vi "Scripting_ConvertBaseClassToSubClass.vi"(0 "BaseClass":refnum<vi>, 1 "NewBaseClass":path=path "C:/Documents and Settings/Micke/Skrivbord/My Computer/B_class/B.lvclass", 2 "SubClassTemplate":path=path "C:/Program/National Instruments/LabVIEW 8.2/resource/Framework/Providers/Endevo/ClassProviders/Provider_EndevoGOOP300/Templates/SubTemplate/SubTemplate.lvclass", 3 "GOOP4Style":bool, 5 "error in (no error)":errorcluster) -> (19 "error out":errorcluster={"status"=TRUE, "code"=1055, "source"="Property Node in Scripting_ConvertBaseClassToSubClass.vi"})   [LabVIEW 2020]
uses:
  <vilib>/Utility/miscctls.llb/LVPositionTypeDef.ctl
  Provider_EndevoGOOP300/EndevoProviderName.ctl
  Provider_EndevoGOOP300/Templates/EndevoTemplateNames.ctl
  Provider_EndevoGOOP400/EndevoG4ProviderName.ctl
  Provider_EndevoGOOP400/Templates/EndevoG4TemplateNames.ctl
  Provider_LvNativeClass/ClassWriterNative_class/ClassWriterNative.lvclass
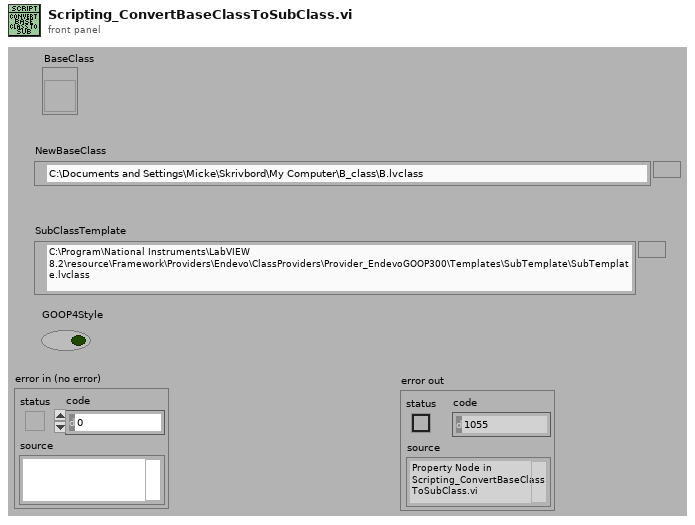
[diagram p1: front panel]
types:
  T1 = cluster{"NewBaseClass":refnum<vi>, "NewBaseCreate ":path, "NewBaseDestroy":path, "NewBaseKernel":path, "NewBaseAttribute":path, "NewBaseClassAttr":path, "NewBaseObjectRef":path, " BaseClass":refnum<vi>, "BaseCreate ":path, "BaseDestroy":path, "BaseKernel":path, "BaseAttribute":path, "BaseClassAttr":path, "BaseClassName":string, "BaseObjectRef":path, "AllBaseClassFiles":path[], "SubNewVi":path, "ObjectRef":refnum<vi>, "BaseNewVi":path, "BaseDeleteVi":path, "SubTemplateKernel":path, "ClassVIs":refnum<vi>[], "SubTemplateClass":refnum<vi>, "BaseTemplateClass":refnum<vi>, "BaseTemplateKernel":path, "BaseAttrRef":refnum<vi>, "BaseClassAttrRef":refnum<vi>, "KernelRef":refnum<vi>, "TemplateVersionUsed":string, "NewBaseNewVI":path, "Singleton":bool, "BaseGetInstance":path, "NewBaseGetInstance":path, "App":refnum<vi>}
  T2 = typedef "LVPositionTypeDef.ctl" = cluster{"Left":i32, "Top":i32}
  T3 = typedef "EndevoTemplateNames.ctl" = enum16{"BaseTemplate", "SubTemplate", "BaseTemplate_4x4x4", "SubTemplate_4x4x4", "SingletonTemplate"}
  T4 = typedef "EndevoProviderName.ctl" = enum16{"EndevoGOOP300"}
  T5 = typedef "EndevoG4TemplateNames.ctl" = enum16{"G4BaseTemplate_Simple_4x4x4", "G4SubTemplate_Simple_4x4x4", "G4BaseTemplate_Simple_6x8x6", "G4SubTemplate_Simple_6x8x6", "G4BaseTemplate_Singleton_4x4x4", "G4SubTemplate_Singleton_4x4x4", "G4BaseTemplate_Singleton_6x8x6", "G4SubTemplate_Singleton_6x8x6", "G4InterfaceTemplate_6x8x6", "G4InterfaceTemplate_4x4x4", "G4BaseTemplate_Simple_5x6x5", "G4BaseTemplate_Singleton_5x6x5", "G4InterfaceTemplate_5x6x5", "G4SubTemplate_Simple_5x6x5", "G4SubTemplate_Singleton_5x6x5"}
  T6 = typedef "EndevoG4ProviderName.ctl" = enum16{"EndevoGOOP400"}
  T7 = cluster{"Major":u16, "Minor":u16, "Fix":u16, "Build":u16}
  T8 = cluster{i32, "WireTermSource":refnum<vi>, "AllWireTerminalDrains":refnum<vi>[]}[]
  T9 = cluster{i32, "AllWireTerminalDrains":refnum<vi>[]}[]
  T10 = typedef "GDSLvCLass_ClassSettingsType.ctl" = cluster{"ClassProviderName":string, "ClassTemplateUsed":string, "ClassTemplateVersion":string, "ClassDescription":string, "PlugIns":T11[], "ConnectorPanePattern":string}
  T11 = typedef "GDSLvClass_PlugIn.ctl" = cluster{"Type":T12, "ID":string, "Version":string, "Path":path, "Name":string, "Data":variant}
  T12 = typedef "GDSLvClass_PlugInTypes.ctl" = enum16{"DesignPattern", "MethodTypes"}
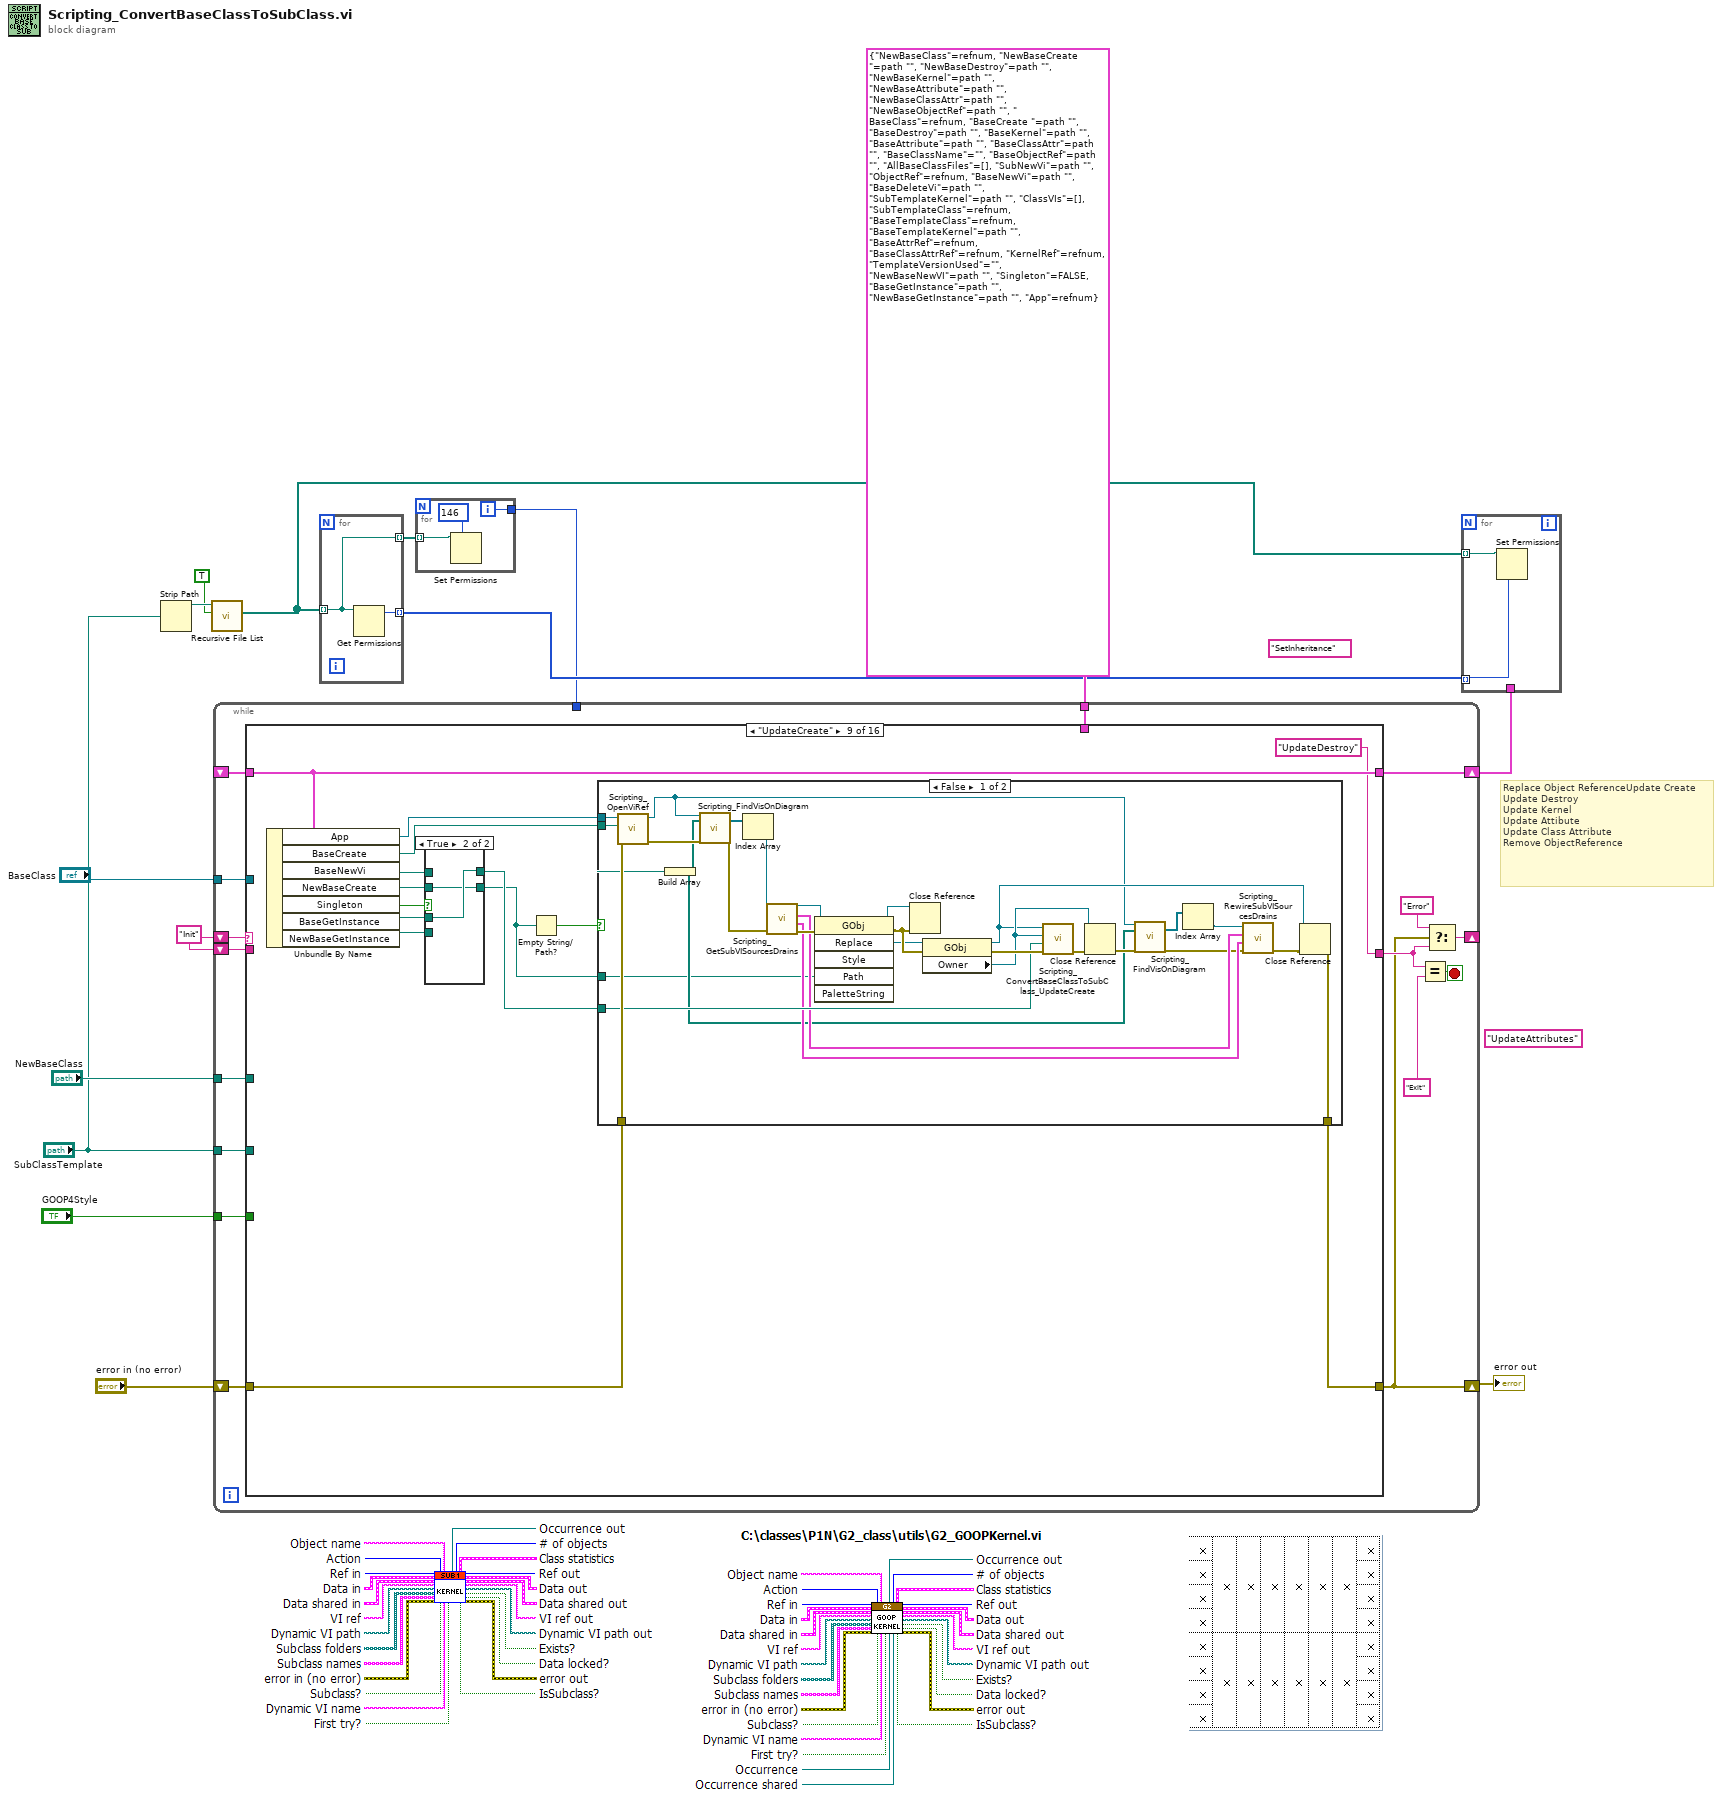
[diagram p0: block diagram]
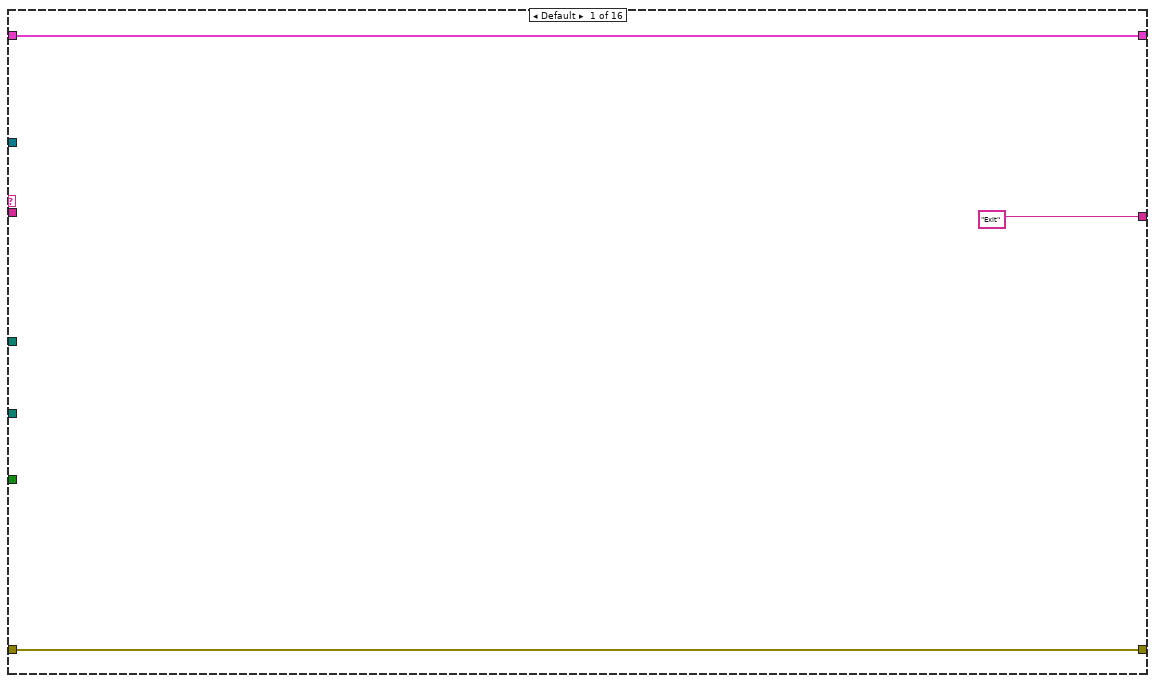
[diagram p2: hidden frame]
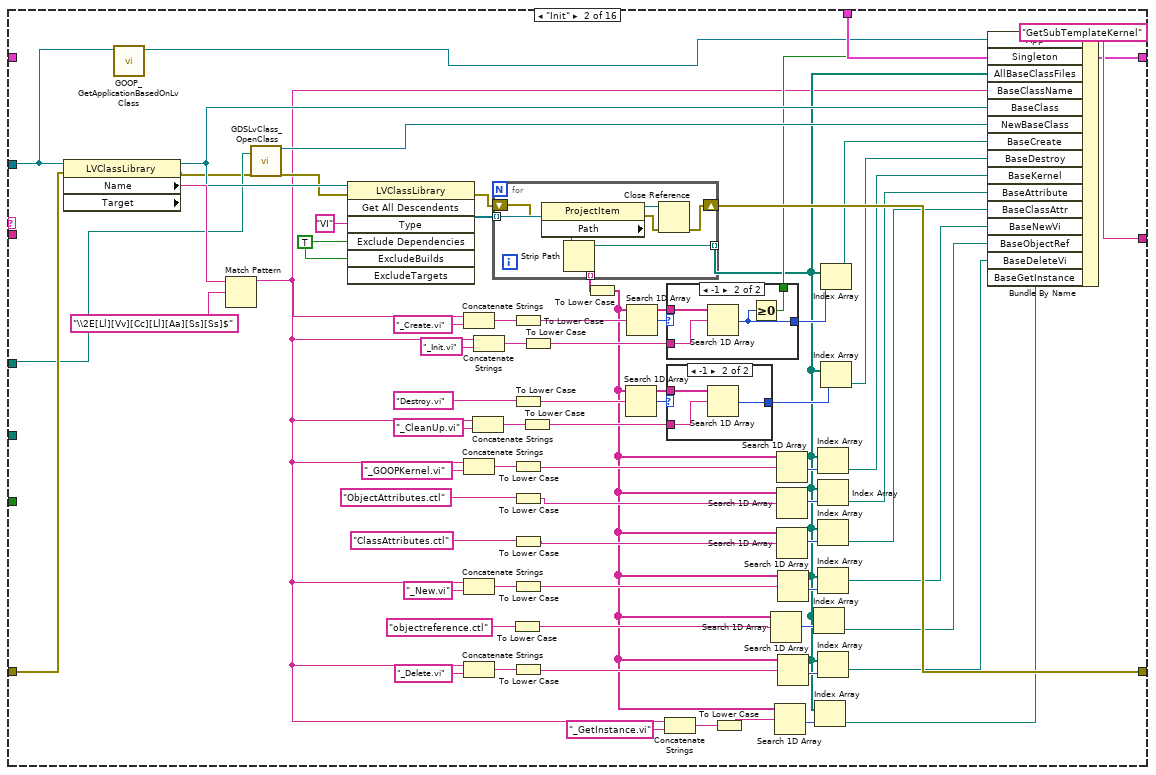
[diagram p3: hidden frame]
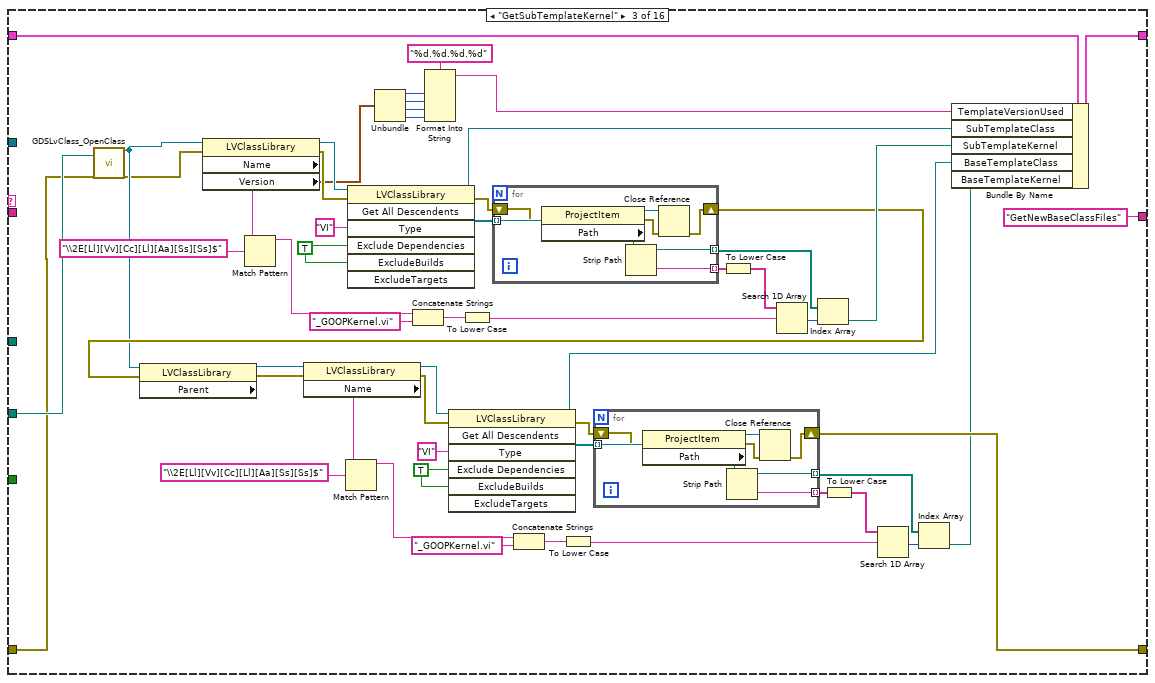
[diagram p6: hidden frame]
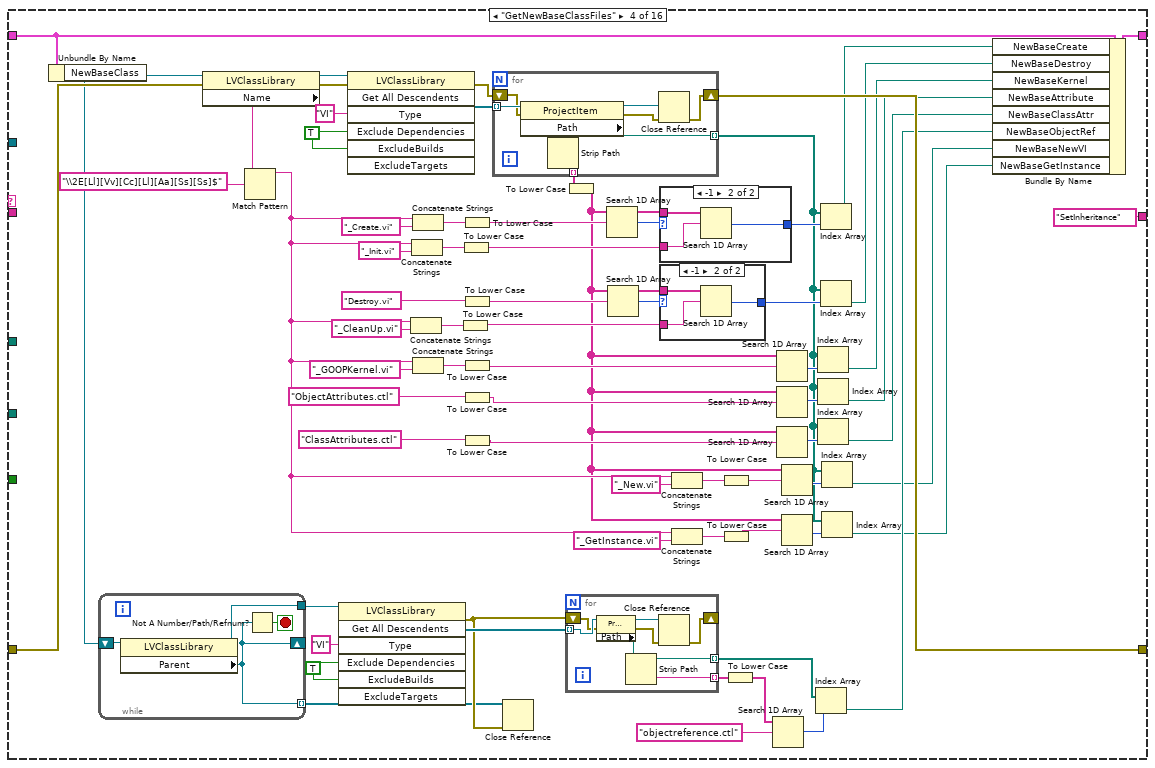
[diagram p7: hidden frame]
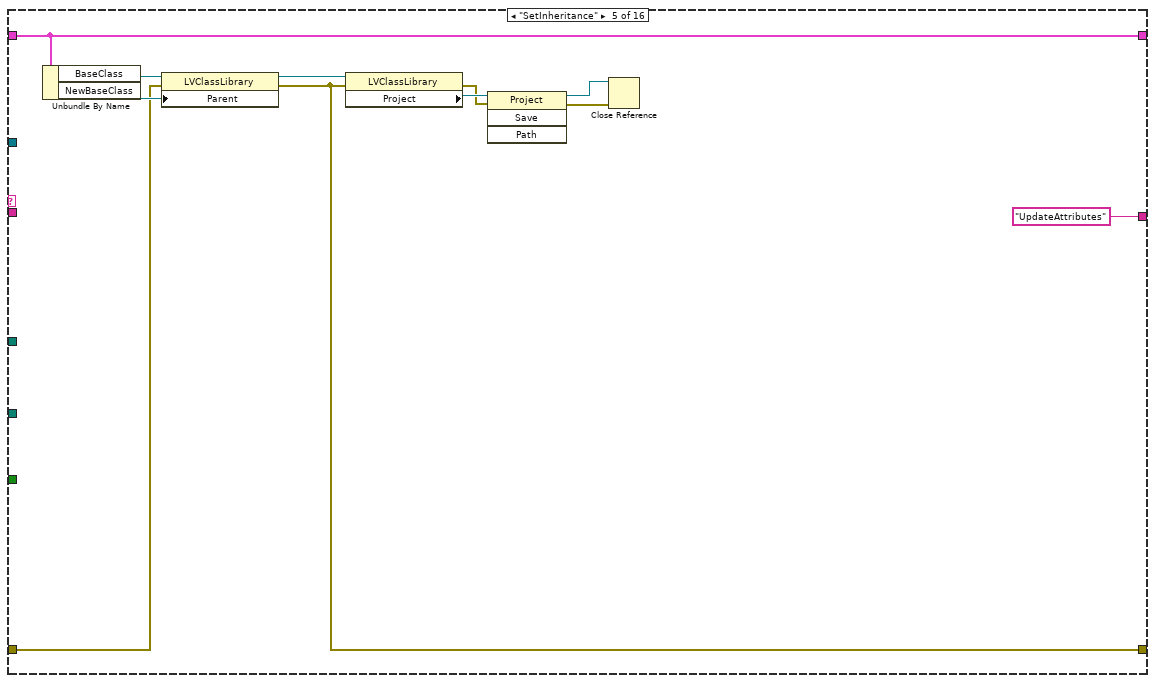
[diagram p10: hidden frame]
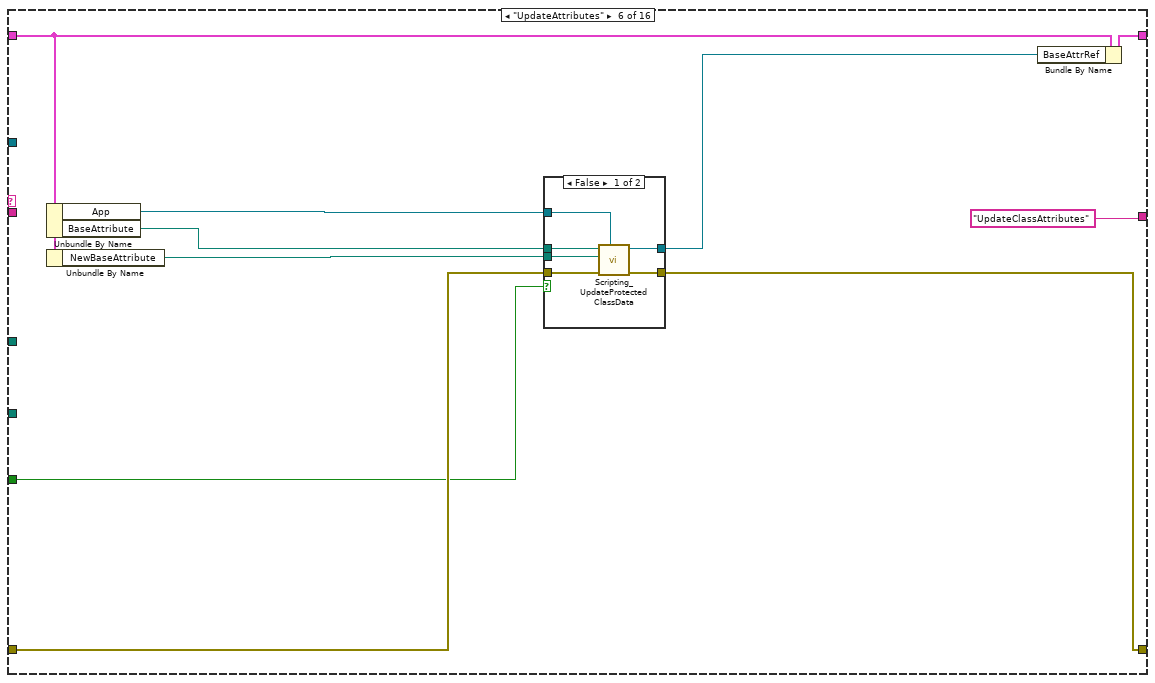
[diagram p11: hidden frame]
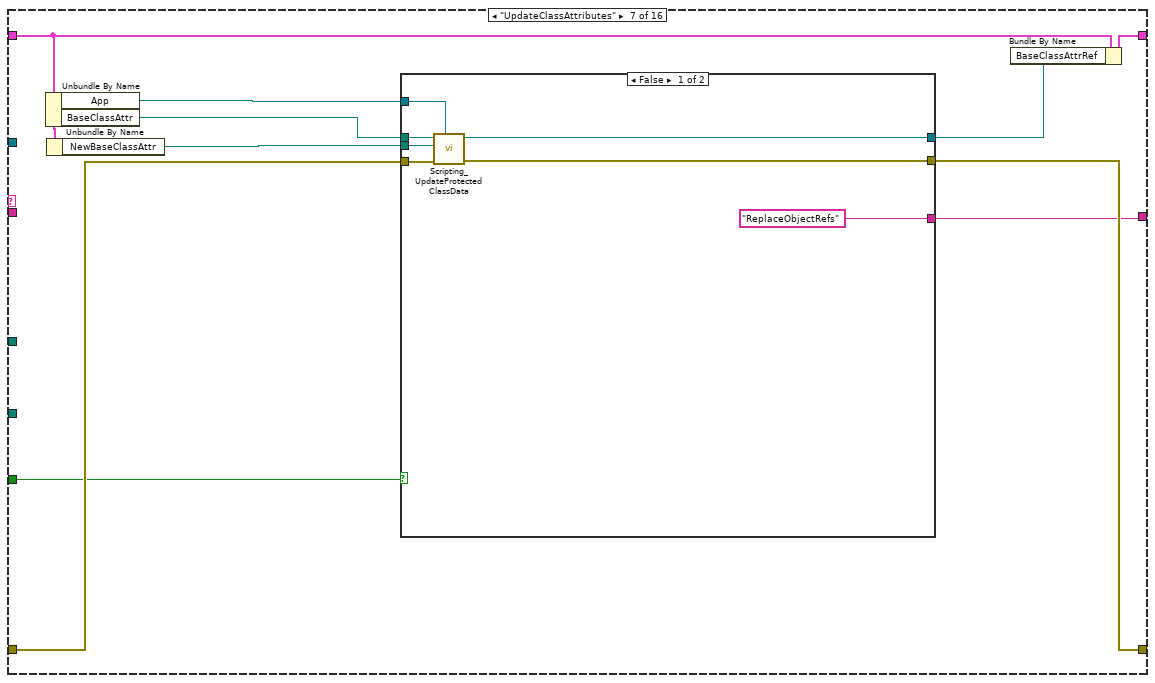
[diagram p13: hidden frame]
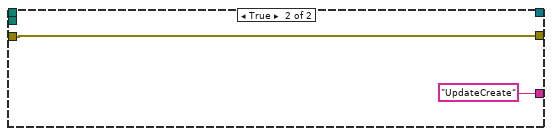
[diagram p14: hidden frame]
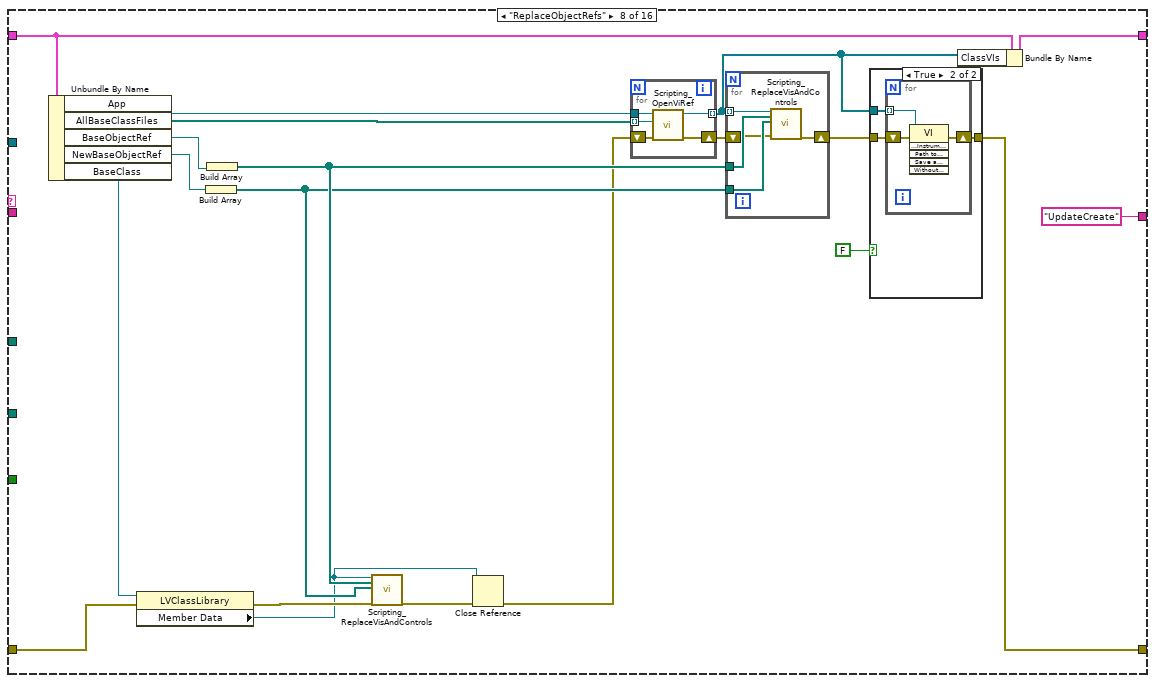
[diagram p15: hidden frame]
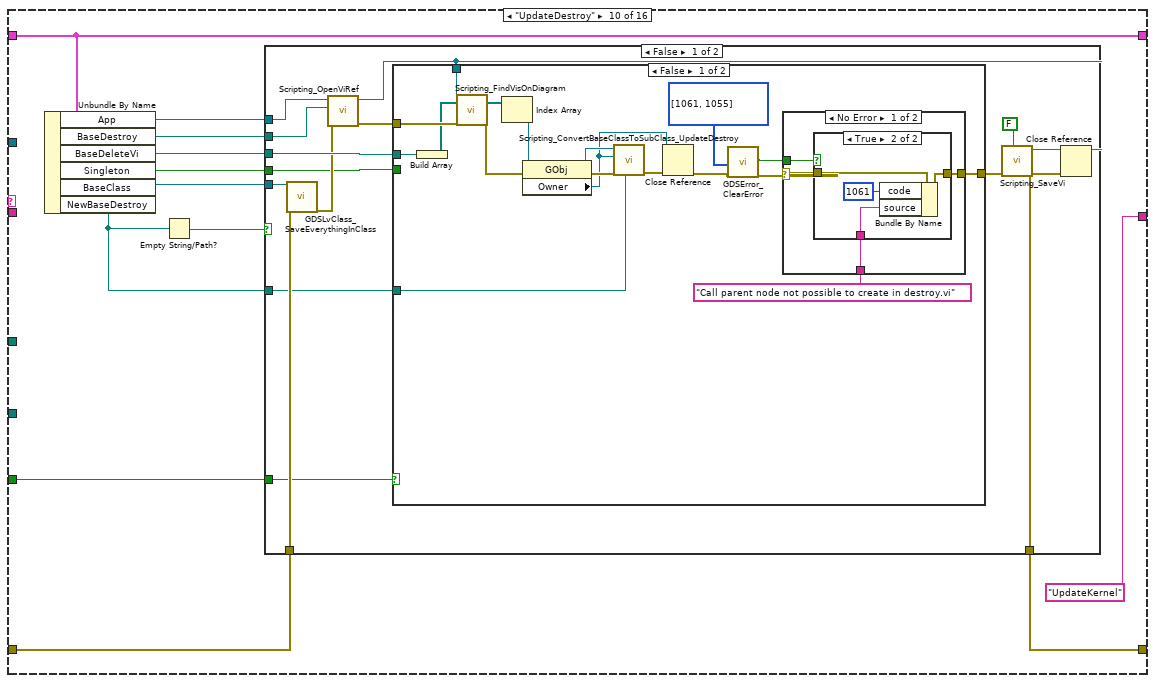
[diagram p19: hidden frame]
diagram:
  (unwired) "SetInheritance"
  (unwired) "UpdateAttributes"
  w10 = "Init"
  # "Replace Object ReferenceUpdate Create\nUpdate Destroy\nUpdate Kernel\nUpdate Attibute\nUpdate Class Attribute\nRemove ObjectReference"
  n1 = Strip Path(path="SubClassTemplate") -> (stripped path=w9:path)  [unwired: 1 out]
  n2 = call <vilib>:"Recursive File List.vi"("Treat LLBs as Folders?"=TRUE, "Folder Path"=w9) -> ("All Files in Dir"=w4:path[])  [unwired: 5 in, 4 out]
  n3 = for {
    tunnel: w4 -> [w16] mode=indexing
    tunnel: [w17] -> w6 mode=indexing
    tunnel: [w16] -> w3 mode=indexing
    n4 = Get Permissions(11:w16) -> (5:w17:i16)  [unwired: 1 in, 4 out]
  }
  n5 = for {
    tunnel: w3 -> [w20] mode=indexing
    tunnel: [w18] -> w5
    i -> [w18]
    n6 = Set Permissions(7:i16 146 ("permissions"), 11:w20) -> ()  [unwired: 3 in, 2 out]
  }
  n7 = while {
    shift-right: [w29] -> w14
    shift-left: "error in (no error)" -> [w36]
    shift-right: [w34] -> _
    shift-left: w10 -> [w35]
    shift-right: [w28] -> w7
    shift-left: _ -> [w27]
    tunnel: "BaseClass" -> [w26]
    tunnel: T1 {"NewBaseClass"=refnum, "NewBaseCreate "=path "", "NewBaseDestroy"=path "", "NewBaseKernel"=path "", "NewBaseAttribute"=path "", "NewBaseClassAttr"=path "", "NewBaseObjectRef"=path "", " BaseClass"=refnum, "BaseCreate "=path "", "BaseDestroy"=path "", "BaseKernel"=path "", "BaseAttribute"=path "", "BaseClassAttr"=path "", "BaseClassName"="", "BaseObjectRef"=path "", "AllBaseClassFiles"=[], "SubNewVi"=path "", "ObjectRef"=refnum, "BaseNewVi"=path "", "BaseDeleteVi"=path "", "SubTemplateKernel"=path "", "ClassVIs"=[], "SubTemplateClass"=refnum, "BaseTemplateClass"=refnum, "BaseTemplateKernel"=path "", "BaseAttrRef"=refnum, "BaseClassAttrRef"=refnum, "KernelRef"=refnum, "TemplateVersionUsed"="", "NewBaseNewVI"=path "", "Singleton"=FALSE, "BaseGetInstance"=path "", "NewBaseGetInstance"=path "", "App"=refnum} -> [w25]
    tunnel: "NewBaseClass" -> [w24]
    tunnel: "SubClassTemplate" -> [w23]
    shift-left: w10 -> [w22]
    tunnel: w5 -> [_]
    tunnel: "GOOP4Style" -> [w21]
    stop <- w33 stop-if-true
    n8 = case shown="\"UpdateCreate\"" w35 {
      tunnel: w36 -> [w39 w77 w137 w236 w299 w310 w325 w347 w387 w429 w503 w643 w673 w715 w760 w770]
      tunnel: [w39 w102 w141 w255 w292 w306 w324 w344 w386 w427 w502 w642 w672 w699 w759 w770] -> w29
      tunnel: ["Exit" "GetSubTemplateKernel" "GetNewBaseClassFiles" "SetInheritance" "UpdateAttributes" "UpdateClassAttributes" w321 "UpdateCreate" "UpdateDestroy" "UpdateKernel" w504 "UpdateClassInfo" "RemoveObjectRef_And_SaveFiles" "UpdateAllDerivedClasses" "CloseReferences" "Exit"] -> w30
      tunnel: [w37 w110 w181 w265 w301 w307 w328 w352 w389 w434 w500 w640 w670 w714 w762 w768] -> w28
      tunnel: w27 -> [w37 _ w169 w237 w301 w308 w329 w353 w389 w434 w501 w640 w670 w714 w762 w768]
      tunnel: w26 -> [_ w41 _ _ _ _ _ _ _ _ _ _ _ _ w758 _]
      tunnel: w25 -> [_ w84 _ _ _ _ _ _ _ _ _ _ _ _ _ _]
      tunnel: w24 -> [_ w65 _ _ _ _ _ _ _ _ _ _ _ _ _ _]
      tunnel: w23 -> [_ _ w166 _ _ _ _ _ _ _ _ _ _ _ _ _]
      tunnel: w22 -> [_ _ _ _ _ _ _ _ _ _ _ _ _ _ _ w769]
      tunnel: w21 -> [_ _ _ _ _ w304 w322 _ _ w428 w499 w644 w663 w697 w757 _]
      frame Default {
      }
      frame "Init" {
        w61 = TRUE ("ExcludeDependencies")
        n9 = property class="LVClassLibrary" props=["Name", "Target"](reference=w41, error in=w77) -> (reference out=w75:refnum<vi>, error out=w64:errorcluster, "Name"=w76:string)  [unwired: 1 out]
        n10 = call "GOOP_GetApplicationBasedOnLvClass.vi"("LVClassLibrary in"=w41) -> ("Application out"=w40:refnum<vi>)  [unwired: 9 in, 1 out]
        n11 = Match Pattern(string=w76, regular expression="\\2E[Ll][Vv][Cc][Ll][Aa][Ss][Ss]$") -> (before substring=w43:string)  [unwired: 1 in, 3 out]
        n12 = call "GDSLvClass_OpenClass.vi"("ClassToOpen"=w65, "error in (no error)"=w64) -> ("LVClass.Open"=w62:refnum<vi>, "error out"=w63:errorcluster)  [unwired: 16 in]
        n13 = invoke class="LVClassLibrary" method="Get All Descendents"(reference=w75, error in=w63, "Type"="VI", "Exclude Dependencies"=w61, "ExcludeBuilds"=w61) -> (error out=w107:errorcluster, "All Descendents"=w108:refnum<vi>[])  [unwired: 2 in, 5 out]
        n14 = Concatenate Strings(w43, "_Create.vi" ("string")) -> (w104:string)
        n15 = Concatenate Strings(w43, "_GOOPKernel.vi" ("string")) -> (w98:string)
        n16 = Concatenate Strings(w43, "_New.vi" ("string")) -> (w81:string)
        n17 = Concatenate Strings(w43, "_Delete.vi" ("string")) -> (w69:string)
        n18 = Concatenate Strings(w43, "_CleanUp.vi" ("string")) -> (w59:string)
        n19 = Concatenate Strings(w43, "_Init.vi" ("string")) -> (w60:string)
        n20 = for {
          tunnel: w108 -> [w127] mode=indexing
          shift-right: [w123] -> w102
          shift-left: w107 -> [w124]
          tunnel: [w122] -> w45 mode=indexing
          tunnel: [w121] -> w105 mode=indexing
          n21 = property class="ProjectItem"(reference=w127, error in=w124) -> (reference out=w126:refnum<vi>, error out=w125:errorcluster, "Path"=w122:path)
          n22 = Strip Path(path=w122) -> (name=w121:string)  [unwired: 1 out]
          n23 = Close Reference(reference=w126, error in (no error)=w125) -> (error out=w123:errorcluster)
        }
        n24 = To Lower Case(string="objectreference.ctl" ("element")) -> (all lower case string=w73:string)
        n25 = To Lower Case(string=w104) -> (all lower case string=w103:string)
        n26 = To Lower Case(string="Destroy.vi") -> (all lower case string=w100:string)
        n27 = To Lower Case(string=w98) -> (all lower case string=w96:string)
        n28 = To Lower Case(string="ObjectAttributes.ctl") -> (all lower case string=w91:string)
        n29 = To Lower Case(string="ClassAttributes.ctl") -> (all lower case string=w88:string)
        n30 = To Lower Case(string=w81) -> (all lower case string=w82:string)
        n31 = To Lower Case(string=w69) -> (all lower case string=w67:string)
        n32 = To Lower Case(string=w59) -> (all lower case string=w57:string)
        n33 = To Lower Case(string=w60) -> (all lower case string=w58:string)
        n34 = To Lower Case(string=w105) -> (all lower case string=w44:string[])
        n35 = Search 1D Array(1D array=w44, element=w100) -> (index of element=w54:i32)  [unwired: 1 in]
        n36 = Search 1D Array(1D array=w44, element=w103) -> (index of element=w56:i32)  [unwired: 1 in]
        n37 = Concatenate Strings(w43, "_GetInstance.vi" ("string")) -> (w48:string)
        n38 = case shown="-1" w56 {
          selector: w56 -> [w116 _]
          tunnel: w44 -> [_ w120]
          tunnel: w58 -> [_ w119]
          tunnel: [w116 w118] -> w55
          tunnel: [_ w117] -> w50
          frame 0, Default {
          }
          frame -1 {
            n39 = Search 1D Array(1D array=w120, element=w119) -> (index of element=w118:i32)  [unwired: 1 in]
            n40 = Greater Or Equal To 0?(x=w118) -> (x >= 0?=w117:bool)
          }
        }
        n41 = case shown="-1" w54 {
          selector: w54 -> [w112 _]
          tunnel: w44 -> [_ w115]
          tunnel: w57 -> [_ w114]
          tunnel: [w112 w113] -> w53
          frame 0, Default {
          }
          frame -1 {
            n42 = Search 1D Array(1D array=w115, element=w114) -> (index of element=w113:i32)  [unwired: 1 in]
          }
        }
        n43 = To Lower Case(string=w48) -> (all lower case string=w46:string)
        n44 = Search 1D Array(1D array=w44, element=w73) -> (index of element=w74:i32)  [unwired: 1 in]
        n45 = Search 1D Array(1D array=w44, element=w46) -> (index of element=w47:i32)  [unwired: 1 in]
        n46 = Search 1D Array(1D array=w44, element=w96) -> (index of element=w95:i32)  [unwired: 1 in]
        n47 = Search 1D Array(1D array=w44, element=w91) -> (index of element=w90:i32)  [unwired: 1 in]
        n48 = Search 1D Array(1D array=w44, element=w88) -> (index of element=w89:i32)  [unwired: 1 in]
        n49 = Search 1D Array(1D array=w44, element=w82) -> (index of element=w79:i32)  [unwired: 1 in]
        n50 = Search 1D Array(1D array=w44, element=w67) -> (index of element=w68:i32)  [unwired: 1 in]
        n51 = Index Array(array=w45, index=w74) -> (element=w71:path)
        n52 = Index Array(array=w45, index=w47) -> (element=w42:path)
        n53 = Index Array(array=w45, index=w95) -> (element=w87:path)
        n54 = Index Array(array=w45, index=w90) -> (element=w86:path)
        n55 = Index Array(array=w45, index=w89) -> (element=w85:path)
        n56 = Index Array(array=w45, index=w79) -> (element=w78:path)
        n57 = Index Array(array=w45, index=w68) -> (element=w66:path)
        n58 = Index Array(array=w45, index=w55) -> (element=w99:path)
        n59 = Index Array(array=w45, index=w53) -> (element=w94:path)
        n60 = Bundle By Name(cluster=w84, "App"=w40, "Singleton"=w50, "AllBaseClassFiles"=w45, "BaseClassName"=w43, "BaseClass"=w75, "NewBaseClass"=w62, "BaseCreate"=w99, "BaseDestroy"=w94, "BaseKernel"=w87, "BaseAttribute"=w86, "BaseClassAttr"=w85, "BaseNewVi"=w78, "BaseObjectRef"=w71, "BaseDeleteVi"=w66, "BaseGetInstance"=w42) -> (w110:T1)
      }
      frame "GetSubTemplateKernel" {
        w135 = TRUE ("ExcludeDependencies")
        w136 = TRUE ("ExcludeDependencies")
        n61 = call "GDSLvClass_OpenClass.vi"("ClassToOpen"=w166, "error in (no error)"=w137) -> ("LVClass.Open"=w159:refnum<vi>, "error out"=w138:errorcluster)  [unwired: 16 in]
        n62 = property class="LVClassLibrary"(reference=w159, error in=w138) -> (reference out=w176:refnum<vi>, error out=w177:errorcluster, "Name"=w168:string, "Version"=w129:T7)
        n63 = Match Pattern(string=w168, regular expression="\\2E[Ll][Vv][Cc][Ll][Aa][Ss][Ss]$") -> (before substring=w165:string)  [unwired: 1 in, 3 out]
        n64 = invoke class="LVClassLibrary" method="Get All Descendents"(reference=w176, error in=w177, "Type"="VI", "Exclude Dependencies"=w135, "ExcludeBuilds"=w135) -> (reference out=w161:refnum<vi>, error out=w178:errorcluster, "All Descendents"=w179:refnum<vi>[])  [unwired: 2 in, 4 out]
        n65 = Unbundle(w129) -> ("Major"=w134:u16, "Minor"=w133:u16, "Fix"=w132:u16, "Build"=w131:u16)
        n66 = Concatenate Strings(w165, "_GOOPKernel.vi" ("string")) -> (w174:string)
        n67 = Format Into String(format string="%d.%d.%d.%d", w134, w133, w132, w131) -> (resulting string=w128:string)  [unwired: 2 in, 1 out]
        n68 = To Lower Case(string=w174) -> (all lower case string=w172:string)
        n69 = for {
          tunnel: w179 -> [w195] mode=indexing
          shift-right: [w191] -> w160
          shift-left: w178 -> [w192]
          tunnel: [w190] -> w164 mode=indexing
          tunnel: [w189] -> w175 mode=indexing
          n70 = property class="ProjectItem"(reference=w195, error in=w192) -> (reference out=w194:refnum<vi>, error out=w193:errorcluster, "Path"=w190:path)
          n71 = Strip Path(path=w190) -> (name=w189:string)  [unwired: 1 out]
          n72 = Close Reference(reference=w194, error in (no error)=w193) -> (error out=w191:errorcluster)
        }
        n73 = property class="LVClassLibrary"(reference=w159, error in=w160) -> (error out=w143:errorcluster, "Parent"=w144:refnum<vi>)  [unwired: 1 out]
        n74 = property class="LVClassLibrary"(reference=w144, error in=w143) -> (reference out=w149:refnum<vi>, error out=w148:errorcluster, "Name"=w155:string)
        n75 = Match Pattern(string=w155, regular expression="\\2E[Ll][Vv][Cc][Ll][Aa][Ss][Ss]$") -> (before substring=w156:string)  [unwired: 1 in, 3 out]
        n76 = invoke class="LVClassLibrary" method="Get All Descendents"(reference=w149, error in=w148, "Type"="VI", "Exclude Dependencies"=w136, "ExcludeBuilds"=w136) -> (reference out=w142:refnum<vi>, error out=w147:errorcluster, "All Descendents"=w146:refnum<vi>[])  [unwired: 2 in, 4 out]
        n77 = Concatenate Strings(w156, "_GOOPKernel.vi" ("string")) -> (w151:string)
        n78 = To Lower Case(string=w151) -> (all lower case string=w153:string)
        n79 = for {
          tunnel: w146 -> [w188] mode=indexing
          shift-right: [w184] -> w141
          shift-left: w147 -> [w185]
          tunnel: [w183] -> w157 mode=indexing
          tunnel: [w182] -> w150 mode=indexing
          n80 = property class="ProjectItem"(reference=w188, error in=w185) -> (reference out=w187:refnum<vi>, error out=w186:errorcluster, "Path"=w183:path)
          n81 = Strip Path(path=w183) -> (name=w182:string)  [unwired: 1 out]
          n82 = Close Reference(reference=w187, error in (no error)=w186) -> (error out=w184:errorcluster)
        }
        n83 = To Lower Case(string=w175) -> (all lower case string=w163:string[])
        n84 = Search 1D Array(1D array=w163, element=w172) -> (index of element=w171:i32)  [unwired: 1 in]
        n85 = Index Array(array=w164, index=w171) -> (element=w170:path)
        n86 = To Lower Case(string=w150) -> (all lower case string=w158:string[])
        n87 = Search 1D Array(1D array=w158, element=w153) -> (index of element=w154:i32)  [unwired: 1 in]
        n88 = Index Array(array=w157, index=w154) -> (element=w140:path)
        n89 = Bundle By Name(cluster=w169, "TemplateVersionUsed"=w128, "SubTemplateClass"=w161, "SubTemplateKernel"=w170, "BaseTemplateClass"=w142, "BaseTemplateKernel"=w140) -> (w181:T1)
      }
      frame "GetNewBaseClassFiles" {
        w221 = TRUE ("ExcludeDependencies")
        w222 = TRUE ("ExcludeDependencies")
        n90 = Unbundle By Name(w237) -> ("NewBaseClass"=w234:refnum<vi>)
        n91 = while {
          shift-right: [w282] -> _
          shift-left: w234 -> [w283]
          tunnel: [w282] -> w204 mode=indexing
          tunnel: [w281] -> w232
          stop <- w284 stop-if-true
          n92 = property class="LVClassLibrary"(reference=w283) -> (reference out=w281:refnum<vi>, "Parent"=w282:refnum<vi>)  [unwired: 1 in, 1 out]
          n93 = Not A Number/Path/Refnum?(number/path/refnum=w282) -> (NaN/Path/Refnum?=w284:bool)
        }
        n94 = property class="LVClassLibrary"(reference=w234, error in=w236) -> (reference out=w260:refnum<vi>, error out=w261:errorcluster, "Name"=w235:string)
        n95 = Match Pattern(string=w235, regular expression="\\2E[Ll][Vv][Cc][Ll][Aa][Ss][Ss]$") -> (before substring=w201:string)  [unwired: 1 in, 3 out]
        n96 = invoke class="LVClassLibrary" method="Get All Descendents"(reference=w232, "Type"="VI", "Exclude Dependencies"=w222, "ExcludeBuilds"=w222) -> (error out=w205:errorcluster, "All Descendents"=w231:refnum<vi>[])  [unwired: 3 in, 5 out]
        n97 = invoke class="LVClassLibrary" method="Get All Descendents"(reference=w260, error in=w261, "Type"="VI", "Exclude Dependencies"=w221, "ExcludeBuilds"=w221) -> (error out=w262:errorcluster, "All Descendents"=w263:refnum<vi>[])  [unwired: 2 in, 5 out]
        n98 = Concatenate Strings(w201, "_CleanUp.vi" ("string")) -> (w210:string)
        n99 = Concatenate Strings(w201, "_Init.vi" ("string")) -> (w211:string)
        n100 = Concatenate Strings(w201, "_Create.vi" ("string")) -> (w257:string)
        n101 = Concatenate Strings(w201, "_GOOPKernel.vi" ("string")) -> (w251:string)
        n102 = To Lower Case(string=w210) -> (all lower case string=w206:string)
        n103 = To Lower Case(string=w211) -> (all lower case string=w207:string)
        n104 = To Lower Case(string=w257) -> (all lower case string=w256:string)
        n105 = To Lower Case(string="Destroy.vi") -> (all lower case string=w253:string)
        n106 = To Lower Case(string=w251) -> (all lower case string=w249:string)
        n107 = To Lower Case(string="ObjectAttributes.ctl") -> (all lower case string=w244:string)
        n108 = To Lower Case(string="ClassAttributes.ctl") -> (all lower case string=w241:string)
        n109 = for {
          tunnel: w263 -> [w291] mode=indexing
          shift-right: [w287] -> w255
          shift-left: w262 -> [w288]
          tunnel: [w286] -> w199 mode=indexing
          tunnel: [w285] -> w258 mode=indexing
          n110 = property class="ProjectItem"(reference=w291, error in=w288) -> (reference out=w290:refnum<vi>, error out=w289:errorcluster, "Path"=w286:path)
          n111 = Strip Path(path=w286) -> (name=w285:string)  [unwired: 1 out]
          n112 = Close Reference(reference=w290, error in (no error)=w289) -> (error out=w287:errorcluster)
        }
        n113 = Close Reference(reference=w204, error in (no error)=w205) -> ()  [unwired: 1 out]
        n114 = To Lower Case(string=w258) -> (all lower case string=w198:string[])
        n115 = for {
          tunnel: w231 -> [w280] mode=indexing
          shift-right: [w276] -> _
          shift-left: w205 -> [w277]
          tunnel: [w275] -> w226 mode=indexing
          tunnel: [w274] -> w230 mode=indexing
          n116 = property class="ProjectItem"(reference=w280, error in=w277) -> (reference out=w279:refnum<vi>, error out=w278:errorcluster, "Path"=w275:path)
          n117 = Strip Path(path=w275) -> (name=w274:string)  [unwired: 1 out]
          n118 = Close Reference(reference=w279, error in (no error)=w278) -> (error out=w276:errorcluster)
        }
        n119 = Search 1D Array(1D array=w198, element=w256) -> (index of element=w215:i32)  [unwired: 1 in]
        n120 = Search 1D Array(1D array=w198, element=w253) -> (index of element=w213:i32)  [unwired: 1 in]
        n121 = case shown="-1" w215 {
          selector: w215 -> [w270 _]
          tunnel: w198 -> [_ w273]
          tunnel: w207 -> [_ w272]
          tunnel: [w270 w271] -> w214
          frame 0, Default {
          }
          frame -1 {
            n122 = Search 1D Array(1D array=w273, element=w272) -> (index of element=w271:i32)  [unwired: 1 in]
          }
        }
        n123 = case shown="-1" w213 {
          selector: w213 -> [w266 _]
          tunnel: w198 -> [_ w269]
          tunnel: w206 -> [_ w268]
          tunnel: [w266 w267] -> w212
          frame 0, Default {
          }
          frame -1 {
            n124 = Search 1D Array(1D array=w269, element=w268) -> (index of element=w267:i32)  [unwired: 1 in]
          }
        }
        n125 = Concatenate Strings(w201, "_New.vi" ("string")) -> (w219:string)
        n126 = Concatenate Strings(w201, "_GetInstance.vi" ("string")) -> (w202:string)
        n127 = To Lower Case(string=w219) -> (all lower case string=w220:string)
        n128 = To Lower Case(string=w202) -> (all lower case string=w197:string)
        n129 = To Lower Case(string=w230) -> (all lower case string=w224:string[])
        n130 = Search 1D Array(1D array=w224, element="objectreference.ctl") -> (index of element=w227:i32)  [unwired: 1 in]
        n131 = Search 1D Array(1D array=w198, element=w249) -> (index of element=w248:i32)  [unwired: 1 in]
        n132 = Search 1D Array(1D array=w198, element=w244) -> (index of element=w243:i32)  [unwired: 1 in]
        n133 = Search 1D Array(1D array=w198, element=w241) -> (index of element=w242:i32)  [unwired: 1 in]
        n134 = Search 1D Array(1D array=w198, element=w220) -> (index of element=w217:i32)  [unwired: 1 in]
        n135 = Search 1D Array(1D array=w198, element=w197) -> (index of element=w200:i32)  [unwired: 1 in]
        n136 = Index Array(array=w226, index=w227) -> (element=w225:path)
        n137 = Index Array(array=w199, index=w248) -> (element=w240:path)
        n138 = Index Array(array=w199, index=w243) -> (element=w239:path)
        n139 = Index Array(array=w199, index=w242) -> (element=w238:path)
        n140 = Index Array(array=w199, index=w214) -> (element=w252:path)
        n141 = Index Array(array=w199, index=w212) -> (element=w247:path)
        n142 = Index Array(array=w199, index=w217) -> (element=w216:path)
        n143 = Index Array(array=w199, index=w200) -> (element=w196:path)
        n144 = Bundle By Name(cluster=w237, "NewBaseCreate"=w252, "NewBaseDestroy"=w247, "NewBaseKernel"=w240, "NewBaseAttribute"=w239, "NewBaseClassAttr"=w238, "NewBaseObjectRef"=w225, "NewBaseNewVI"=w216, "NewBaseGetInstance"=w196) -> (w265:T1)
      }
      frame "SetInheritance" {
        n145 = Unbundle By Name(w301) -> ("BaseClass"=w302:refnum<vi>, "NewBaseClass"=w300:refnum<vi>)
        n146 = property class="LVClassLibrary"(reference=w302, error in=w299, "Parent"=w300) -> (reference out=w297:refnum<vi>, error out=w292:errorcluster)
        n147 = property class="LVClassLibrary"(reference=w297, error in=w292) -> (error out=w293:errorcluster, "Project"=w296:refnum<vi>)  [unwired: 1 out]
        n148 = invoke class="Project" method="Save"(reference=w296, error in=w293) -> (reference out=w294:refnum<vi>, error out=w295:errorcluster)  [unwired: 2 in, 2 out]
        n149 = Close Reference(reference=w294, error in (no error)=w295) -> ()  [unwired: 1 out]
      }
      frame "UpdateAttributes" {
        n150 = Unbundle By Name(w308) -> ("App"=w303:refnum<vi>, "BaseAttribute"=w311:path)
        n151 = Unbundle By Name(w308) -> ("NewBaseAttribute"=w309:path)
        n152 = case shown="False" w304 {
          tunnel: w311 -> [w318 _]
          tunnel: w310 -> [w317 w319]
          tunnel: w309 -> [w316 _]
          tunnel: [w315 w319] -> w306
          tunnel: [w314 _] -> w305
          tunnel: w303 -> [w313 _]
          frame False {
            n153 = call "Scripting_UpdateProtectedClassData.vi"("AppRef"=w313, "error in (no error)"=w317, "NewBaseAttribute"=w316, "BaseAttribute"=w318) -> ("error out"=w315:errorcluster, "BaseAttributeReference"=w314:refnum<vi>)  [unwired: 6 in]
          }
          frame True {
          }
        }
        n154 = Bundle By Name(cluster=w308, "BaseAttrRef"=w305) -> (w307:T1)
      }
      frame "UpdateClassAttributes" {
        n155 = Unbundle By Name(w329) -> ("App"=w320:refnum<vi>, "BaseClassAttr"=w327:path)
        n156 = Unbundle By Name(w329) -> ("NewBaseClassAttr"=w326:path)
        n157 = case shown="False" w322 {
          tunnel: w327 -> [w336 _]
          tunnel: w326 -> [w335 _]
          tunnel: w325 -> [w334 w338]
          tunnel: [w333 w338] -> w324
          tunnel: [w332 _] -> w323
          tunnel: ["ReplaceObjectRefs" "UpdateCreate"] -> w321
          tunnel: w320 -> [w330 _]
          frame False {
            n158 = call "Scripting_UpdateProtectedClassData.vi"("AppRef"=w330, "error in (no error)"=w334, "NewBaseAttribute"=w335, "BaseAttribute"=w336) -> ("error out"=w333:errorcluster, "BaseAttributeReference"=w332:refnum<vi>)  [unwired: 6 in]
          }
          frame True {
          }
        }
        n159 = Bundle By Name(cluster=w329, "BaseClassAttrRef"=w323) -> (w328:T1)
      }
      frame "ReplaceObjectRefs" {
        n160 = Unbundle By Name(w353) -> ("App"=w339:refnum<vi>, "AllBaseClassFiles"=w350:path[], "BaseObjectRef"=w357:path, "NewBaseObjectRef"=w356:path, "BaseClass"=w348:refnum<vi>)
        n161 = property class="LVClassLibrary"(reference=w348, error in=w347) -> (error out=w346:errorcluster, "Member Data"=w343:refnum<vi>)  [unwired: 1 out]
        n162 = Build Array(w356) -> (w354:path[])
        n163 = Build Array(w357) -> (w355:path[])
        n164 = call "Scripting_ReplaceVisAndControls.vi"("ViRef"=w343, "OldVIsAndControls"=w355, "NewVIsAndControls"=w354, "error in (no error)"=w346) -> ("error out"=w340:errorcluster)  [unwired: 14 in, 1 out]
        n165 = Close Reference(reference=w343, error in (no error)=w340) -> (error out=w345:errorcluster)
        n166 = for {
          shift-right: [w370] -> w342
          shift-left: w345 -> [w369]
          tunnel: w350 -> [w368] mode=indexing
          tunnel: [w367] -> w349 mode=indexing
          tunnel: w339 -> [w366]
          n167 = call "Scripting_OpenViRef.vi"("error in"=w369, "ViPath/ViName/Viref"=w368, "AppRef"=w366) -> ("error out"=w370:errorcluster, "vi reference"=w367:refnum<vi>)  [unwired: 6 in, 1 out]
        }
        n168 = for {
          shift-right: [w375] -> w351
          shift-left: w342 -> [w372]
          tunnel: w355 -> [w374]
          tunnel: w354 -> [w373]
          tunnel: w349 -> [w371] mode=indexing
          n169 = call "Scripting_ReplaceVisAndControls.vi"("ViRef"=w371, "OldVIsAndControls"=w374, "NewVIsAndControls"=w373, "error in (no error)"=w372) -> ("error out"=w375:errorcluster)  [unwired: 14 in, 1 out]
        }
        n170 = case shown="True" FALSE {
          tunnel: w351 -> [w359 w362]
          tunnel: w349 -> [_ w361]
          tunnel: [w359 w360] -> w344
          frame False {
          }
          frame True {
            n171 = for {
              shift-right: [w364] -> w360
              shift-left: w362 -> [w365]
              tunnel: w361 -> [w363] mode=indexing
              n172 = invoke class="VI" method="Save.Instrument"(reference=w363, error in=w365) -> (error out=w364:errorcluster)  [unwired: 4 in, 5 out]
            }
          }
        }
        n173 = Bundle By Name(cluster=w353, "ClassVIs"=w349) -> (w352:T1)
      }
      frame "UpdateCreate" {
        n174 = Unbundle By Name(w389) -> ("App"=w379:refnum<vi>, "BaseCreate"=w388:path, "BaseNewVi"=w384:path, "NewBaseCreate"=w383:path, "Singleton"=w385:bool, "BaseGetInstance"=w381:path, "NewBaseGetInstance"=w380:path)
        n175 = case shown="True" w385 {
          tunnel: w384 -> [w420 _]
          tunnel: w383 -> [w419 w421]
          tunnel: [w420 w422] -> w382
          tunnel: [w419 w421] -> w378
          tunnel: w381 -> [_ w422]
          tunnel: w380 -> [_ _]
          frame False {
          }
          frame True {
          }
        }
        n176 = Empty String/Path?(string/path=w378) -> (empty?=w376:bool)
        n177 = case shown="False" w376 {
          tunnel: w388 -> [w417 _]
          tunnel: w387 -> [w416 w418]
          tunnel: [w407 w418] -> w386
          tunnel: w382 -> [w406 _]
          tunnel: w379 -> [w391 _]
          tunnel: w378 -> [w390 _]
          frame False {
            n178 = call "Scripting_OpenViRef.vi"("error in"=w416, "ViPath/ViName/Viref"=w417, "AppRef"=w391) -> ("error out"=w415:errorcluster, "vi reference"=w396:refnum<vi>)  [unwired: 6 in, 1 out]
            n179 = Build Array(w406) -> (w395:path[])
            n180 = call "Scripting_FindVisOnDiagram.vi"("ViRef"=w396, "VIsToSerachFor/ViName"=w395, "error in (no error)"=w415) -> ("VisFound"=w414:refnum<vi>[], "error out"=w405:errorcluster)  [unwired: 15 in]
            n181 = Index Array(array=w414) -> (element=w404:refnum<vi>)  [unwired: 1 in]
            n182 = call "Scripting_GetSubVISourcesDrains.vi"("error in (no error)"=w405, "SubVIIn"=w404) -> ("error out"=w403:errorcluster, "DrainsSources"=w399:T8, "SourceDrains"=w400:T9, "SubVIOut"=w402:refnum<vi>)  [unwired: 6 in]
            n183 = invoke class="GObj" method="Replace"(reference=w402, error in=w403, "Path"=w390) -> (reference out=w413:refnum<vi>, error out=w412:errorcluster, "Replace"=w411:refnum<vi>)  [unwired: 3 in, 3 out]
            n184 = Close Reference(reference=w413, error in (no error)=w412) -> ()  [unwired: 1 out]
            n185 = property class="GObj"(reference=w411, error in=w412) -> (reference out=w398:refnum<vi>, error out=w410:errorcluster, "Owner"=w409:refnum<vi>)
            n186 = call "Scripting_ConvertBaseClassToSubClass_UpdateCreate.vi"("error in (no error)"=w410, "NewViPath"=w406, "Diagram"=w409, "NewBaseCreate"=w398) -> ("error out"=w408:errorcluster)  [unwired: 7 in]
            n187 = Close Reference(reference=w409, error in (no error)=w408) -> (error out=w397:errorcluster)
            n188 = call "Scripting_FindVisOnDiagram.vi"("ViRef"=w396, "VIsToSerachFor/ViName"=w395, "error in (no error)"=w397) -> ("VisFound"=w392:refnum<vi>[], "error out"=w393:errorcluster)  [unwired: 15 in]
            n189 = Index Array(array=w392) -> (element=w394:refnum<vi>)  [unwired: 1 in]
            n190 = call "Scripting_RewireSubVISourcesDrains.vi"("error in"=w393, "DrainsSources"=w399, "SourceDrains"=w400, "SubVIIn"=w394) -> ("error out"=w401:errorcluster)  [unwired: 7 in]
            n191 = Close Reference(reference=w398, error in (no error)=w401) -> (error out=w407:errorcluster)
          }
          frame True {
          }
        }
      }
      frame "UpdateDestroy" {
        n192 = Unbundle By Name(w434) -> ("App"=w425:refnum<vi>, "BaseDestroy"=w433:path, "BaseDeleteVi"=w432:path, "Singleton"=w426:bool, "BaseClass"=w430:refnum<vi>, "NewBaseDestroy"=w424:path)
        n193 = Empty String/Path?(string/path=w424) -> (empty?=w423:bool)
        n194 = case shown="False" w423 {
          tunnel: w433 -> [w449 _]
          tunnel: w432 -> [w447 _]
          tunnel: w430 -> [w444 _]
          tunnel: w429 -> [w443 w498]
          tunnel: w428 -> [w440 _]
          tunnel: [w439 w498] -> w427
          tunnel: w426 -> [w437 _]
          tunnel: w425 -> [w436 _]
          tunnel: w424 -> [w435 _]
          frame False {
            n195 = call "GDSLvClass_SaveEverythingInClass.vi"("ClassRefIn"=w444, "error in"=w443) -> ("error out"=w441:errorcluster)  [unwired: 16 in, 1 out]
            n196 = call "Scripting_OpenViRef.vi"("error in"=w441, "ViPath/ViName/Viref"=w449, "AppRef"=w436) -> ("error out"=w448:errorcluster, "vi reference"=w445:refnum<vi>)  [unwired: 6 in, 1 out]
            n197 = case shown="False" w440 {
              tunnel: w448 -> [w467 w480]
              tunnel: w447 -> [w462 _]
              tunnel: w445 -> [w458 w481]
              tunnel: [w452 w483] -> w442
              tunnel: w435 -> [w451 w482]
              tunnel: w437 -> [_ w478]
              frame False {
                n198 = Build Array(w462) -> (w466:path[])
                n199 = call "Scripting_FindVisOnDiagram.vi"("ViRef"=w458, "VIsToSerachFor/ViName"=w466, "error in (no error)"=w467) -> ("VisFound"=w465:refnum<vi>[], "error out"=w461:errorcluster)  [unwired: 15 in]
                n200 = Index Array(array=w465) -> (element=w459:refnum<vi>)  [unwired: 1 in]
                n201 = property class="GObj"(reference=w459, error in=w461) -> (reference out=w464:refnum<vi>, error out=w463:errorcluster, "Owner"=w450:refnum<vi>)
                n202 = call "Scripting_ConvertBaseClassToSubClass_UpdateDestroy.vi"("BaseClassDestroyViPath"=w451, "error in (no error)"=w463, "Diagram"=w450, "DeleteViRef"=w464) -> ("error out"=w460:errorcluster)  [unwired: 7 in]
                n203 = Close Reference(reference=w450, error in (no error)=w460) -> (error out=w457:errorcluster)
                n204 = call "GDSError_ClearError.vi"("codes"=i32[] [1061, 1055], "error in (no error)"=w457) -> ("Cleared?"=w454:bool, "error out"=w455:errorcluster)  [unwired: 16 in]
                n205 = case shown="No Error" w455 {
                  selector: w455 -> [w470 w477]
                  tunnel: w454 -> [w471 _]
                  tunnel: "Call parent node not possible to create in destroy.vi" ("source") -> [w469 _]
                  tunnel: [w468 w477] -> w452
                  frame No Error {
                    n206 = case shown="True" w471 {
                      tunnel: w470 -> [w472 w476]
                      tunnel: w469 -> [_ w474]
                      tunnel: [w472 w473] -> w468
                      frame False {
                      }
                      frame True {
                        n207 = Bundle By Name(cluster=w476, "code"=1061, "source"=w474) -> (w473:errorcluster)
                      }
                    }
                  }
                  frame Error {
                  }
                }
              }
              frame True {
                n208 = call "Scripting_G4ConvertBaseClassToSubClass_UpdateDestroy.vi"("BaseClassDestroyViPath"=w482, "error in (no error)"=w480, "Singleton"=w478, "ViRef"=w481) -> ("error out"=w479:errorcluster)  [unwired: 7 in]
                n209 = call "GDSError_ClearError.vi"("codes"=i32[] [1061, 1055], "error in (no error)"=w479) -> ("Cleared?"=w485:bool, "error out"=w486:errorcluster)  [unwired: 16 in]
                n210 = case shown="No Error" w486 {
                  selector: w486 -> [w490 w497]
                  tunnel: w485 -> [w491 _]
                  tunnel: "Call parent node not possible to create in destroy.vi" ("source") -> [w489 _]
                  tunnel: [w488 w497] -> w483
                  frame No Error {
                    n211 = case shown="True" w491 {
                      tunnel: w490 -> [w492 w496]
                      tunnel: w489 -> [_ w494]
                      tunnel: [w492 w493] -> w488
                      frame False {
                      }
                      frame True {
                        n212 = Bundle By Name(cluster=w496, "code"=1061, "source"=w494) -> (w493:errorcluster)
                      }
                    }
                  }
                  frame Error {
                  }
                }
              }
            }
            n213 = call "Scripting_SaveVi.vi"("ForceResaving(False)"=FALSE, "error in (no error)"=w442, "VIRefToSaveIn"=w445) -> ("error out"=w439:errorcluster, "VIRefToSaveOut"=w438:refnum<vi>)  [unwired: 7 in]
            n214 = Close Reference(reference=w438, error in (no error)=w439) -> ()  [unwired: 1 out]
          }
          frame True {
          }
        }
      }
      frame "UpdateKernel" {
        n215 = case shown="False" w499 {
          tunnel: ["UpdateClassInfo" "UpdateNEWVI"] -> w504
          tunnel: w503 -> [w558 w624]
          tunnel: [w510 w625] -> w502
          tunnel: w501 -> [w506 w623]
          tunnel: [w528 w622] -> w500
          frame False {
            n216 = Unbundle By Name(w506) -> ("App"=w505:refnum<vi>, "BaseKernel"=w579:path, "SubTemplateKernel"=w525:path)
            n217 = call "Scripting_OpenViRef.vi"("error in"=w558, "ViPath/ViName/Viref"=w579, "AppRef"=w505) -> ("error out"=w578:errorcluster, "vi reference"=w569:refnum<vi>)  [unwired: 6 in, 1 out]
            n218 = property class="VI"(reference=w569, error in=w578) -> (reference out=w564:refnum<vi>, error out=w527:errorcluster, "Diagram"=w567:refnum<vi>)
            n219 = Unbundle By Name(w506) -> ("SubTemplateClass"=w513:refnum<vi>, "BaseClass"=w512:refnum<vi>)
            n220 = property class="TopLvlDiag"(reference=w567, error in=w527) -> (reference out=w561:refnum<vi>, error out=w566:errorcluster, "AllObjs[]"=w565:refnum<vi>[])
            n221 = Unbundle By Name(w506) -> ("BaseAttribute"=w546:path, "BaseClassAttr"=w541:path, "BaseTemplateKernel"=w533:path, "NewBaseKernel"=w531:path)
            n222 = for {
              tunnel: w566 -> [w614]
              tunnel: w565 -> [w615] mode=indexing
              tunnel: [w614] -> w563
              n223 = invoke class="GObj" method="Delete"(reference=w615, error in=w614) -> (reference out=w616:refnum<vi>)  [unwired: 1 in, 2 out]
              n224 = Close Reference(reference=w616) -> ()  [unwired: 1 in, 1 out]
            }
            n225 = invoke class="VI" method="BD.Remove Bad Wires"(reference=w564, error in=w563) -> (reference out=w560:refnum<vi>, error out=w526:errorcluster)  [unwired: 1 in, 1 out]
            n226 = call "Scripting_OpenViRef.vi"("error in"=w526, "ViPath/ViName/Viref"=w525, "AppRef"=w505) -> ("error out"=w523:errorcluster, "vi reference"=w522:refnum<vi>)  [unwired: 6 in, 1 out]
            n227 = invoke class="VI" method="Fake Exec State"(reference=w522, "state"=2 ("State")) -> (reference out=w521:refnum<vi>)  [unwired: 2 in, 3 out]
            n228 = property class="VI"(reference=w521, error in=w523) -> (reference out=w518:refnum<vi>, error out=w577:errorcluster, "Diagram"=w574:refnum<vi>)
            n229 = invoke class="TopLvlDiag" method="Select All"(reference=w574, error in=w577) -> (reference out=w575:refnum<vi>, error out=w576:errorcluster)  [unwired: 1 in, 1 out]
            n230 = invoke class="TopLvlDiag" method="Copy Selection"(reference=w575, error in=w576) -> (reference out=w519:refnum<vi>, error out=w562:errorcluster)  [unwired: 1 in, 1 out]
            n231 = invoke class="TopLvlDiag" method="Paste"(reference=w561, error in=w562, "Pos"=T2 {"Left"=50, "Top"=50} ("Position")) -> (reference out=w539:refnum<vi>, error out=w540:errorcluster)  [unwired: 1 in, 2 out]
            n232 = invoke class="App" method="Clipboard.Empty"(error in=w540) -> (error out=w520:errorcluster)  [unwired: 2 in, 2 out]
            n233 = property class="VI"(reference=w560, error in=w520) -> (error out=w571:errorcluster, "Panel"=w572:refnum<vi>)  [unwired: 1 out]
            n234 = Close Reference(reference=w539) -> ()  [unwired: 1 in, 1 out]
            n235 = property class="Pnl"(reference=w572, error in=w571) -> (reference out=w538:refnum<vi>, error out=w570:errorcluster, "Controls[]"=w536:refnum<vi>[])
            n236 = Build Array(w531) -> (w530:path[])
            n237 = Build Array(w533) -> (w532:path[])
            n238 = Close Reference(reference=w519, error in (no error)=w520) -> (error out=w537:errorcluster)
            n239 = Close Reference(reference=w518, error in (no error)=w537) -> ()  [unwired: 1 out]
            n240 = for {
              tunnel: w536 -> [w617] mode=indexing
              shift-right: [w619] -> w568
              shift-left: w570 -> [w620]
              tunnel: [w618] -> w514 mode=indexing
              n241 = property class="Ctl"(reference=w617, error in=w620) -> (error out=w619:errorcluster, "Label.Text"=w618:string)  [unwired: 1 out]
            }
            n242 = property class="VI"(reference=w569, error in=w568) -> (reference out=w507:refnum<vi>, error out=w559:errorcluster, "ConPane"=w534:refnum<vi>)
            n243 = Search 1D Array(1D array=w514, element="Dynamic VI path" ("Id")) -> (index of element=w508:i32)  [unwired: 1 in]
            n244 = case shown="Default" w508 {
              tunnel: [string[] ["Data in", "Data out", "Action", "Ref in", "Ref out", "Data locked?", "error out", "error in (no error)", "Subclass?", "Object name", "Exists?", "Data shared out", "Data shared in", "Subclass names", "Class name", "Probe in", "Class statistics", "IsSubclass?", "Misc", "# of objects", "Occurrence out", "Occurrence", "Occurrence shared", "Probe out"] ("Array") string[] ["Data in", "Data out", "Action", "Ref in", "Ref out", "Data locked?", "error out", "error in (no error)", "Subclass?", "Object name", "Exists?", "Data shared out", "Data shared in", "Subclass folders", "Subclass names", "Dynamic VI name", "VI ref out", "Dynamic VI path", "Dynamic VI path out", "VI ref", "Class statistics", "IsSubclass?", "First try?", "# of objects", "Occurrence out", "Occurrence", "Occurrence shared"] ("Array")] -> w517
              tunnel: [i32[] [1, 21, 8, 0, 20, 26, 27, 7, 9, 10, 25, 22, 2, 6, 11, 3, 18, 19, 13, 16, 14, 15, 17, 23] i32[] [1, 21, 8, 0, 20, 26, 27, 7, 9, 10, 25, 22, 2, 5, 6, 11, 23, 4, 24, 3, 18, 19, 13, 16, 14, 15, 17]] -> w516
              frame -1 {
              }
              frame Default {
              }
            }
            n245 = for {
              tunnel: w514 -> [w604] mode=indexing
              tunnel: w534 -> [w613]
              tunnel: w517 -> [w606]
              tunnel: w536 -> [w607] mode=indexing
              tunnel: w516 -> [w611]
              shift-right: [w608] -> w535
              shift-left: w559 -> [w609]
              n246 = Search and Replace String(replace all?=TRUE ("replace all? (F)"), input string=w604, search string="\n", replace string=" " ("replace string (\"\")")) -> (result string=w603:string)  [unwired: 4 in, 3 out]
              n247 = Search 1D Array(1D array=w606, element=w603) -> (index of element=w612:i32)  [unwired: 1 in]
              n248 = Index Array(array=w611, index=w612) -> (element=w610:i32)
              n249 = invoke class="ConPane" method="AssignCtrlToTerm"(reference=w613, error in=w609, "Control"=w607, "TermIdx"=w610) -> (error out=w608:errorcluster)  [unwired: 1 in, 4 out]
            }
            n250 = Close Reference(reference=w534, error in (no error)=w535) -> ()  [unwired: 1 out]
            n251 = Search 1D Array(1D array=w514, element="Data in" ("Label.Text")) -> (index of element=w557:i32)  [unwired: 1 in]
            n252 = Search 1D Array(1D array=w514, element="Data out" ("Label.Text")) -> (index of element=w553:i32)  [unwired: 1 in]
            n253 = Search 1D Array(1D array=w514, element="Data shared in" ("Label.Text")) -> (index of element=w552:i32)  [unwired: 1 in]
            n254 = Search 1D Array(1D array=w514, element="Data shared out" ("Label.Text")) -> (index of element=w551:i32)  [unwired: 1 in]
            n255 = Index Array(array=w536, index=w557) -> (element=w555:refnum<vi>)
            n256 = Index Array(array=w536, index=w553) -> (element=w547:refnum<vi>)
            n257 = Index Array(array=w536, index=w552) -> (element=w543:refnum<vi>)
            n258 = Index Array(array=w536, index=w551) -> (element=w542:refnum<vi>)
            n259 = invoke class="Ctl" method="Replace"(reference=w555, error in=w535, "Path"=w546) -> (error out=w554:errorcluster)  [unwired: 3 in, 5 out]
            n260 = invoke class="Ctl" method="Replace"(reference=w547, error in=w554, "Path"=w546) -> (error out=w544:errorcluster)  [unwired: 3 in, 5 out]
            n261 = Close Reference(reference=w538) -> ()  [unwired: 1 in, 1 out]
            n262 = invoke class="Ctl" method="Replace"(reference=w543, error in=w544, "Path"=w541) -> (error out=w545:errorcluster)  [unwired: 3 in, 5 out]
            n263 = Bundle By Name(cluster=w506, "KernelRef"=w507) -> (w528:T1)
            n264 = invoke class="Ctl" method="Replace"(reference=w542, error in=w545, "Path"=w541) -> (error out=w509:errorcluster)  [unwired: 3 in, 5 out]
            n265 = case shown="-1" w508 {
              tunnel: w507 -> [_ w594]
              tunnel: w509 -> [w581 w593]
              tunnel: [w581 w592] -> w511
              tunnel: w513 -> [_ w589]
              tunnel: w512 -> [_ w588]
              frame Default {
              }
              frame -1 {
                n266 = property class="LVClassLibrary"(reference=w589) -> ("Path"=w585:path)  [unwired: 1 in, 2 out]
                n267 = property class="LVClassLibrary"(reference=w588) -> ("Path"=w587:path)  [unwired: 1 in, 2 out]
                n268 = call <vilib>:"Get File Extension.vi"("file"=w585) -> ("filename without extension"=w584:string)  [unwired: 6 in, 4 out]
                n269 = Concatenate Strings(w584, ".ctl" ("string")) -> (w583:string)
                n270 = Build Path(base path=w585, name or relative path=w583) -> (appended path=w586:path)
                n271 = Build Array(w586) -> (w591:path[])
                n272 = Build Array(w587) -> (w590:path[])
                n273 = call "Scripting_ReplaceVisAndControls.vi"("ViRef"=w594, "OldVIsAndControls"=w591, "NewVIsAndControls"=w590, "error in (no error)"=w593) -> ("error out"=w592:errorcluster)  [unwired: 14 in, 1 out]
              }
            }
            n274 = call "Scripting_ReplaceVisAndControls.vi"("ViRef"=w507, "OldVIsAndControls"=w532, "NewVIsAndControls"=w530, "error in (no error)"=w511) -> ("error out"=w529:errorcluster)  [unwired: 14 in, 1 out]
            n275 = for {
              tunnel: w536 -> [w600] mode=indexing
              shift-right: [w599] -> w510
              shift-left: w529 -> [w599]
              n276 = Close Reference(reference=w600, error in (no error)=w599) -> ()  [unwired: 1 out]
            }
          }
          frame True {
            n277 = disable-structure shown="Enabled" {
              disable-tunnel: [w634 w635] -> w625
              disable-tunnel: w624 -> [w632 w635]
              disable-tunnel: w623 -> [w629 w636]
              disable-tunnel: [w627 w636] -> w622
              frame Disabled {
                n278 = Unbundle By Name(w629) -> ("BaseKernel"=w633:path, "SubTemplateKernel"=w631:path)
                n279 = call "Scripting_OpenViRef.vi"("error in"=w632, "ViPath/ViName/Viref"=w633) -> ("error out"=w630:errorcluster, "vi reference"=w628:refnum<vi>)  [unwired: 7 in, 1 out]
                n280 = call "Scripting_UpdateViFromTemplate.vi"("ViRef"=w628, "TemplateVI(Path or Ref)"=w631, "error in (no error)"=w630) -> ("TemplateVersionUsed"=w626:string, "error out"=w634:errorcluster)  [unwired: 15 in]
                n281 = Bundle By Name(cluster=w629, "KernelRef"=w628, "TemplateVersionUsed"=w626) -> (w627:T1)
              }
              frame Enabled {
              }
            }
          }
        }
      }
      frame "UpdateNEWVI" {
        n282 = Unbundle By Name(w640) -> ("App"=w639:refnum<vi>, "BaseNewVi"=w645:path, "NewBaseNewVI"=w638:path)
        n283 = Empty String/Path?(string/path=w638) -> (empty?=w637:bool)
        n284 = case shown="True" w637 {
          tunnel: w645 -> [w651 _]
          tunnel: w644 -> [w650 _]
          tunnel: w643 -> [w649 w658]
          tunnel: [w648 w658] -> w642
          tunnel: w639 -> [w647 _]
          tunnel: w638 -> [w646 _]
          frame False {
            n285 = case shown="True" w650 {
              tunnel: w649 -> [w652 w657]
              tunnel: [w652 w656] -> w648
              tunnel: w651 -> [_ w655]
              tunnel: w646 -> [_ w654]
              tunnel: w647 -> [_ w653]
              frame False {
              }
              frame True {
                n286 = call "Scripting_UpdateNewVI.vi"("NewVI Ref or Path"=w655, "BaseClassNewVI Ref or Path(If empty the No base class will be used)"=w654, "error in (no error)"=w657, "AppRef"=w653) -> ("error out"=w656:errorcluster)  [unwired: 15 in]
              }
            }
          }
          frame True {
          }
        }
      }
      frame "UpdateClassInfo" {
        n287 = Unbundle By Name(w670) -> ("TemplateVersionUsed"=w666:string, "BaseClass"=w674:refnum<vi>)
        n288 = property class="LVClassLibrary"(reference=w674, error in=w673) -> (reference out=w669:refnum<vi>, error out=w668:errorcluster, "Description"=w675:string)
        n289 = call "GDSLvClass_ReadClassType.vi"("Class Refnum In"=w669, "error in (no error)"=w668) -> ("Class Refnum Out"=w659:refnum<vi>, "ClassSettings"=w662:T10, "error out"=w667:errorcluster)  [unwired: 15 in]
        n290 = Unbundle By Name(w662) -> ("ClassTemplateUsed"=w661:string)
        n291 = call "GOOP_ClassTemplateSplit.vi"("ClassItemRefIn"=w659, "FullClassTemplate"=w661) -> ("StandardTemplate"=w660:string)  [unwired: 12 in, 1 out]
        n292 = case shown="True" w663 {
          tunnel: [w679 w687] -> w665
          tunnel: [w678 w686] -> w664
          tunnel: w660 -> [w677 w689]
          frame False {
            n293 = Scan From String(input string=w677, default 1=EndevoTemplateNames."BaseTemplate" ("TemplateNames")) -> (output 1=w682:T3)  [unwired: 3 in, 3 out]
            n294 = case shown="\"BaseTemplate_4x4x4\"" w682 {
              tunnel: [EndevoTemplateNames."SubTemplate" ("TemplateNames") EndevoTemplateNames."SubTemplate_4x4x4" ("TemplateNames")] -> w681
              frame "BaseTemplate", Default {
              }
              frame "BaseTemplate_4x4x4" {
              }
            }
            n295 = Format Into String(EndevoProviderName."EndevoGOOP300" ("ProviderName")) -> (resulting string=w679:string)  [unwired: 3 in, 1 out]
            n296 = Format Into String(w681) -> (resulting string=w678:string)  [unwired: 3 in, 1 out]
          }
          frame True {
            n297 = Scan From String(input string=w689, default 1=EndevoG4TemplateNames."G4SubTemplate_Simple_4x4x4" ("TemplateNames")) -> (output 1=w691:T5)  [unwired: 3 in, 3 out]
            n298 = case shown="\"G4BaseTemplate_Singleton_6x8x6\"" w691 {
              tunnel: [EndevoG4TemplateNames."G4SubTemplate_Simple_4x4x4" ("TemplateNames") EndevoG4TemplateNames."G4SubTemplate_Simple_6x8x6" ("TemplateNames") EndevoG4TemplateNames."G4SubTemplate_Singleton_4x4x4" ("TemplateNames") EndevoG4TemplateNames."G4SubTemplate_Singleton_6x8x6" ("TemplateNames")] -> w692
              frame "G4BaseTemplate_Simple_4x4x4", Default {
              }
              frame "G4BaseTemplate_Simple_6x8x6" {
              }
              frame "G4BaseTemplate_Singleton_4x4x4" {
              }
              frame "G4BaseTemplate_Singleton_6x8x6" {
              }
            }
            n299 = Format Into String(EndevoG4ProviderName."EndevoGOOP400" ("ProviderName")) -> (resulting string=w687:string)  [unwired: 3 in, 1 out]
            n300 = Format Into String(w692) -> (resulting string=w686:string)  [unwired: 3 in, 1 out]
          }
        }
        n301 = Bundle By Name(cluster=w662, "ClassTemplateVersion"=w666, "ClassDescription"=w675, "ClassProviderName"=w665, "ClassTemplateUsed"=w664) -> (w676:T10)
        n302 = call "GDSLvClass_StoreClassType.vi"("Class Refnum In"=w659, "ClassSettings"=w676, "error in (no error)"=w667) -> ("error out"=w672:errorcluster)  [unwired: 15 in, 1 out]
      }
      frame "RemoveObjectRef_And_SaveFiles" {
        w698 = i32[] [1040, 1035] ("codes")
        n303 = Unbundle By Name(w714) -> ("BaseClass"=w706:refnum<vi>, "BaseObjectRef"=w712:path)
        n304 = Unbundle By Name(w714) -> ("ClassVIs"=w711:refnum<vi>[], "BaseAttrRef"=w709:refnum<vi>, "BaseClassAttrRef"=w708:refnum<vi>, "KernelRef"=w707:refnum<vi>)
        n305 = Build Array (concatenate)(w711, w709, w708, w707) -> (w710:refnum<vi>[])
        n306 = for {
          tunnel: w710 -> [w747] mode=indexing
          shift-right: [w748] -> w705
          shift-left: w715 -> [w749]
          n307 = Not A Number/Path/Refnum?(number/path/refnum=w747) -> (NaN/Path/Refnum?=w746:bool)
          n308 = case shown="True" w746 {
            tunnel: w749 -> [w754 w756]
            tunnel: [w752 w756] -> w748
            tunnel: w747 -> [w750 _]
            frame False {
              n309 = call "Scripting_SaveVi.vi"("ForceResaving(False)"=FALSE, "error in (no error)"=w754, "VIRefToSaveIn"=w750) -> ("error out"=w753:errorcluster, "VIRefToSaveOut"=w755:refnum<vi>)  [unwired: 7 in]
              n310 = Close Reference(reference=w755, error in (no error)=w753) -> (error out=w752:errorcluster)
            }
            frame True {
            }
          }
        }
        n311 = invoke class="LVClassLibrary" method="Save"(reference=w706, error in=w705) -> (reference out=w703:refnum<vi>, error out=w704:errorcluster)  [unwired: 2 in, 2 out]
        n312 = case shown="False" w697 {
          tunnel: w712 -> [w726 _]
          tunnel: w704 -> [w722 w745]
          tunnel: w703 -> [w721 w744]
          tunnel: [w720 w744] -> w702
          tunnel: [w719 w745] -> w701
          tunnel: w698 -> [w718 _]
          frame False {
            n313 = property class="LVClassLibrary"(reference=w721, error in=w722) -> (reference out=w720:refnum<vi>, error out=w725:errorcluster, "Children[]"=w727:refnum<vi>[])
            n314 = call "GDSError_ClearError.vi"("codes"=w718, "error in (no error)"=w725) -> ("error out"=w724:errorcluster)  [unwired: 16 in, 1 out]
            n315 = for {
              tunnel: w727 -> [w737] mode=indexing
              tunnel: w726 -> [w735]
              shift-right: [w729] -> w723
              shift-left: w724 -> [w731]
              n316 = property class="ProjectItem"(reference=w737, error in=w731) -> (reference out=w733:refnum<vi>, error out=w732:errorcluster, "Path"=w736:path)
              n317 = Equal?(x=w735, y=w736) -> (x = y?=w734:bool)
              n318 = case shown="True" w734 {
                tunnel: w733 -> [w738 w743]
                tunnel: [w739 w742] -> w730
                tunnel: w732 -> [w739 w740]
                tunnel: [w738 w741] -> w728
                frame False {
                }
                frame True {
                  n319 = invoke class="ProjectItem" method="Delete"(reference=w743, error in=w740) -> (reference out=w741:refnum<vi>, error out=w742:errorcluster)  [unwired: 1 in, 1 out]
                }
              }
              n320 = Close Reference(reference=w728, error in (no error)=w730) -> (error out=w729:errorcluster)
            }
            n321 = call "GDSError_ClearError.vi"("codes"=w718, "error in (no error)"=w723) -> ("error out"=w719:errorcluster)  [unwired: 16 in, 1 out]
          }
          frame True {
          }
        }
        n322 = call "GDSLvClass_SaveEverythingInClass.vi"("ClassRefIn"=w702, "error in"=w701) -> ("error out"=w700:errorcluster)  [unwired: 16 in, 1 out]
        n323 = call "GDSError_ClearError.vi"("codes"=w698, "error in (no error)"=w700) -> ("error out"=w699:errorcluster)  [unwired: 16 in, 1 out]
        n324 = case shown="False" w697 {
          tunnel: w712 -> [w717 _]
          tunnel: w699 -> [w716 _]
          frame False {
            n325 = Delete(path (use dialog)=w717, error in=w716) -> ()  [unwired: 3 in, 3 out]
          }
          frame True {
          }
        }
      }
      frame "UpdateAllDerivedClasses" {
        n326 = case shown="False" w757 {
          tunnel: w760 -> [w765 w766]
          tunnel: [w764 w766] -> w759
          tunnel: w758 -> [w763 _]
          frame False {
            n327 = call "Scripting_UpdateDerivedClasses.vi"("ClassRef"=w763, "error in (no error)"=w765) -> ("error out"=w764:errorcluster)  [unwired: 17 in]
          }
          frame True {
          }
        }
      }
      frame "CloseReferences", "Error" {
        n328 = call "GDSError_LogErrorInformation.vi"("State"=w769, "LocalVariableData"=w768, "error in (no error)"=w770) -> ()  [unwired: 16 in, 1 out]
        n329 = Unbundle By Name(w768) -> ("NewBaseClass"=w774:refnum<vi>, "SubTemplateClass"=w772:refnum<vi>, "BaseTemplateClass"=w771:refnum<vi>, "App"=w767:refnum<vi>)
        n330 = Close Reference(reference=w772) -> ()  [unwired: 1 in, 1 out]
        n331 = Close Reference(reference=w771) -> ()  [unwired: 1 in, 1 out]
        n332 = Close Reference(reference=w774) -> ()  [unwired: 1 in, 1 out]
        n333 = Close Reference(reference=w767) -> ()  [unwired: 1 in, 1 out]
      }
    }
    n334 = Equal?(x=w30, y="Exit") -> (x = y?=w33:bool)
    n335 = Select(t="Error", s=w29, f=w30) -> (s? t:f=w34:string)
  }
  "error out" <- w14
  n336 = for {
    tunnel: w4 -> [w776] mode=indexing
    tunnel: w6 -> [w775] mode=indexing
    tunnel: w7 -> [_]
    n337 = Set Permissions(7:w775, 11:w776) -> ()  [unwired: 3 in, 2 out]
  }
